vi "DSS-test-read_r140.vi"(8 "error in":errorcluster) -> (0 "error out":errorcluster)   [LabVIEW 2020, in "DSS-Tests.lvlib"]
doc: "Caraya test of RFH-read-R140 (needs Excel) on water-start.xlsx: length, first and last element of every array of Common Format and R140 data against their golden file."
uses:
  DSS-Tests.lvlib
  <vilib>/addons/_JKI Toolkits/Caraya/classes/Test/Test.lvclass
  Reflector/RFH-Reflection_File_Handler.lvlib
  <vilib>/addons/_JKI Toolkits/Caraya/classes/Assert/Assert.lvclass
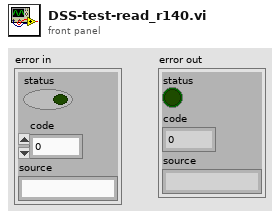
[diagram p1: front panel]
types:
  T1 = typedef "RFH-Reflection_File_Handler.lvlib/RFH-R140_data_format.ctl" = cluster{"Frequency":dbl[], "Permativity'":dbl[], "Permativity''":dbl[], "Q [S/m]":dbl[], "Tan":dbl[], "Reflection R":dbl[], "Reflection I":dbl[]}
  T2 = typedef "RFH-Reflection_File_Handler.lvlib/RFH-common_data_format.ctl" = cluster{"Frequency":dbl[], "Reflection'":dbl[], "Reflection''":dbl[], "Permativity'":dbl[], "Permativity''":dbl[], "Conductivity":dbl[], "Loss Tangent":dbl[], "Resistance":dbl[], "Reactance":dbl[]}
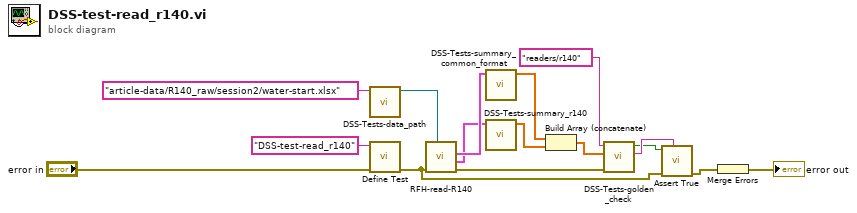
[diagram p0: block diagram]
diagram:
  n1 = call "DSS-Tests-data_path.vi"("relative path"="article-data/R140_raw/session2/water-start.xlsx") -> ("path"=w5:path)  [unwired: 10 in]
  n2 = call <vilib>:"Define Test.vi"("error in (no error)"="error in", "Label (VI Title)"="DSS-test-read_r140") -> ("error out"=w3:errorcluster)  [unwired: 8 in, 1 out]
  n3 = call "RFH-read-R140.vi"("file path (dialog if empty)"=w5, "error in (no error)"=w3) -> ("error out"=w6:errorcluster, "R140 data"=w7:T1, "Common Format"=w8:T2)  [unwired: 7 in]
  n4 = call "DSS-Tests-summary_common_format.vi"("Common Format"=w8) -> ("summary"=w9:dbl[])  [unwired: 10 in]
  n5 = call "DSS-Tests-summary_r140.vi"("R140 data"=w7) -> ("summary"=w10:dbl[])  [unwired: 10 in]
  n6 = Build Array (concatenate)(w9, w10) -> (w11:dbl[])
  n7 = call "DSS-Tests-golden_check.vi"("error in"=w6, "actual"=w11, "golden name"="readers/r140") -> ("message"=w14:string, "pass"=w13:bool)  [unwired: 6 in, 1 out]
  n8 = call <vilib>:"Assert True.vi"("Label"=w14, "error in (no error)"=w3, "True?"=w13) -> ("error out"=w15:errorcluster)  [unwired: 7 in, 1 out]
  n9 = Merge Errors(w15) -> (→"error out":errorcluster)
